vi "VI Template Name--constant.vi"() -> (3 "VI Template Name":string)   [LabVIEW 2026]
doc: "This constant defines the name of the VI template in the main project directory."
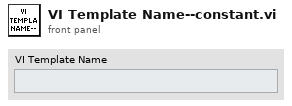
[diagram p1: front panel]
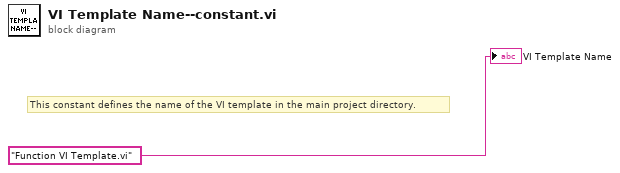
[diagram p0: block diagram]
diagram:
  # "This constant defines the name of the VI template in the main project directory."
  "VI Template Name" <- "Function VI Template.vi"
